vi "Result_Calculate.vi"(8 "error in (no error)":errorcluster={"status"=FALSE, "code"=0, "source"="\"\""}, 10 "resolved measurements":string, 11 "Formula definition":string) -> (0 "error out":errorcluster={"status"=FALSE, "code"=0, "source"="\"\""}, 2 "status ok":bool, 3 "Typed calculated result":string)   [LabVIEW 2026]
doc: "INTENT: Calculate acceptance values. LOGIC: Run supported arithmetic/comparison with units and missing-data policy; produce pass/fail/incomplete."
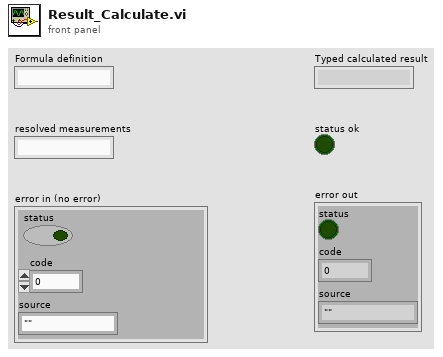
[diagram p1: front panel]
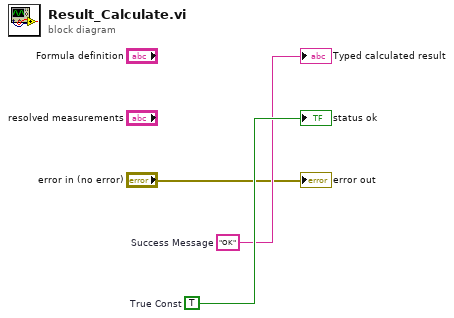
[diagram p0: block diagram]
diagram:
  w3 = TRUE  # True Const
  w2 = "OK"  # Success Message
  "Typed calculated result" <- w2
  "status ok" <- w3
  "error out" <- "error in (no error)"
